vi "RemoteVI Send Overlay.vi"(0 "clients":T2(array[cluster]), 1 "state":T1, 2 "period":dbl=50.0, 5 "overlay popups":T4(array[cluster]), 7 "geo":T3, 9 "d":cluster{"dx":i32, "dy":i32}) -> (4 "clients out":T2(array[cluster]), 6 "state out":T1)   [LabVIEW 2020, in "RemoteVI.lvlib"]
doc: "The OVERLAY part of one server loop iteration (docs\\protocol.md section 3.2). While a popup is open or one was (state.message not empty, to clear it), at most every period ms and only while a client is connected, each popup is captured and PNG-encoded at its LOGICAL position = window position minus (frame origin + d), NOT clipped to the panel, bottom-most first (RemoteVI Encode Popups.vi); RemoteVI Overlay Encode.vi builds the message and it is written to every client (RemoteVI Write To Clients.vi, 500 ms) only when it differs from state.message - an empty OVERLAY when the last popup has closed. state holds the last message, the last frame (sent to a client that connects while a popup is open) - both reset to empty once no popup is open - and the tick count of the last check."
uses:
  RemoteVI.lvlib
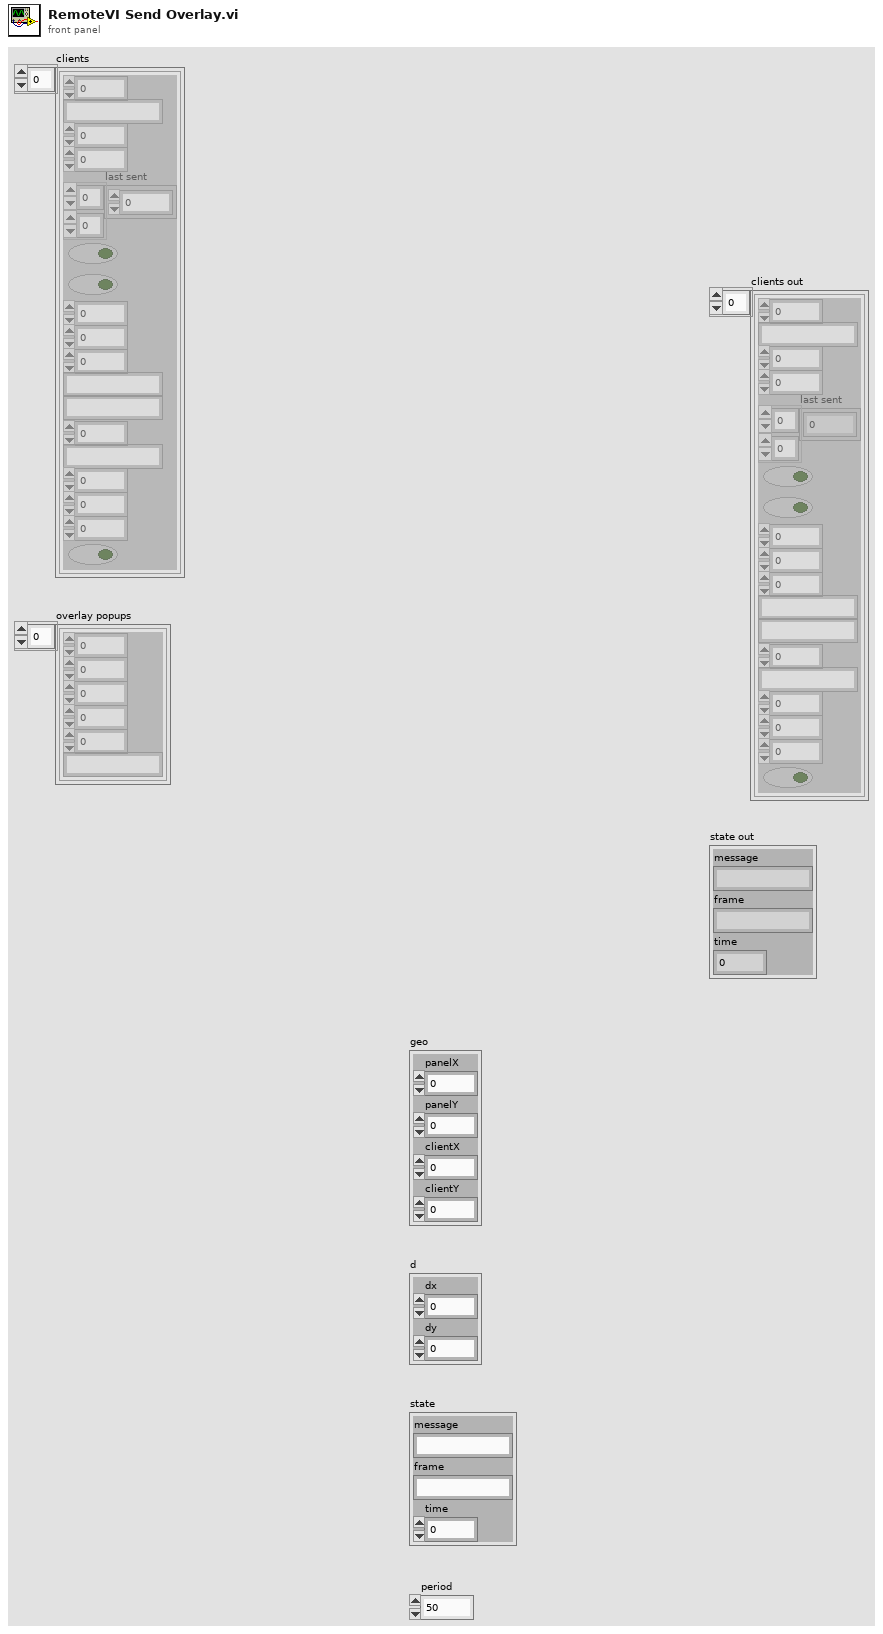
[diagram p1: front panel]
types:
  T1 = cluster{"message":string, "frame":string, "time":u32}
  T2 = cluster{"connection":u32, "rx buffer":string, "seq":u32, "acked":u32, "last sent":u32[][], "tracking":bool, "closed":bool, "mods":u8, "mods set":u8, "popup since":u32, "windows sent":string, "window frames":cluster{"id":u64, "pixels":u32[][]}[], "key window":u64, "address":string, "since":dbl, "last input":dbl, "bytes":dbl, "view only":bool}[]
  T3 = cluster{"panelX":i32, "panelY":i32, "clientX":i32, "clientY":i32}
  T4 = cluster{"hwnd":u64, "x":i32, "y":i32, "w":i32, "h":i32, "class":string}[]
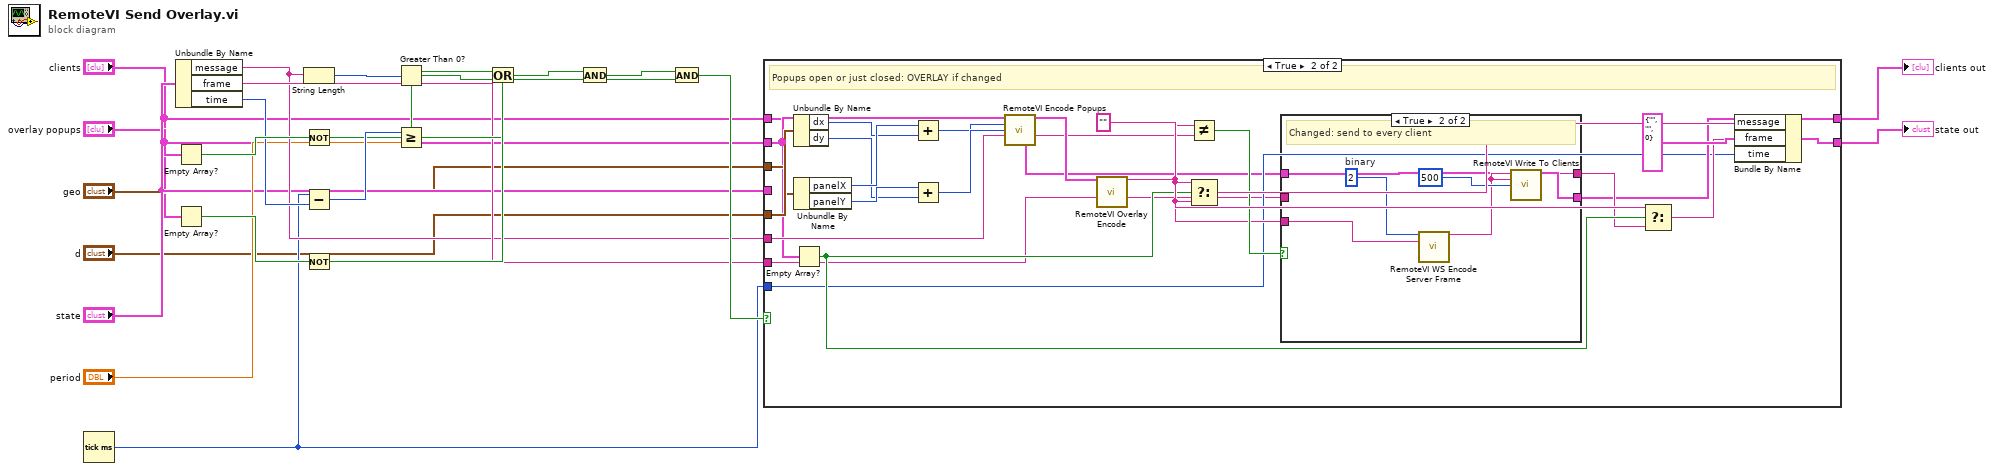
[diagram p0: block diagram]
diagram:
  n1 = Tick Count (ms)() -> (millisecond timer value=w7:u32)
  n2 = Unbundle By Name("state") -> ("message"=w8:string, "frame"=w9:string, "time"=w10:u32)
  n3 = Empty Array?(array="overlay popups") -> (empty?=w13:bool)
  n4 = Empty Array?(array="clients") -> (empty?=w18:bool)
  n5 = String Length(string=w8) -> (length=w11:i32)
  n6 = Not(x=w13) -> (.not. x?=w14:bool)
  n7 = Subtract(x=w7, y=w10) -> (x-y=w16:u32)
  n8 = Not(x=w18) -> (.not. x?=w19:bool)
  n9 = Greater Than 0?(x=w11) -> (x > 0?=w12:bool)
  n10 = Greater Or Equal?(x=w16, y="period") -> (x >= y?=w17:bool)
  n11 = Or(x=w14, y=w12) -> (x .or. y?=w15:bool)
  n12 = And(x=w15, y=w17) -> (x .and. y?=w20:bool)
  n13 = And(x=w20, y=w19) -> (x .and. y?=w21:bool)
  n14 = case shown="True" w21 {
    tunnel: "clients" -> [w24 w26]
    tunnel: "overlay popups" -> [_ w27]
    tunnel: "geo" -> [_ w28]
    tunnel: "state" -> [w25 _]
    tunnel: "d" -> [_ w32]
    tunnel: w8 -> [_ w29]
    tunnel: w9 -> [_ w30]
    tunnel: w7 -> [_ w31]
    tunnel: [w24 w42] -> w22
    tunnel: [w25 w49] -> w23
    frame False {
    }
    frame True {
      w45 = ""
      # "Popups open or just closed: OVERLAY if changed"
      n15 = Unbundle By Name(w32) -> ("dx"=w33:i32, "dy"=w34:i32)
      n16 = Unbundle By Name(w28) -> ("panelX"=w35:i32, "panelY"=w36:i32)
      n17 = Empty Array?(array=w27) -> (empty?=w44:bool)
      n18 = Add(x=w35, y=w33) -> (x+y=w37:i32)
      n19 = Add(x=w36, y=w34) -> (x+y=w38:i32)
      n20 = call "RemoteVI Encode Popups.vi"("popups"=w27, "origin x"=w37, "origin y"=w38) -> ("overlay popups"=w39:cluster{"x":i16, "y":i16, "png":string}[])  [unwired: 12 in]
      n21 = call "RemoteVI Overlay Encode.vi"("popups"=w39) -> ("message"=w40:string)  [unwired: 14 in]
      n22 = Not Equal?(x=w40, y=w29) -> (x != y?=w41:bool)
      n23 = Select(t=w45, s=w44, f=w40) -> (s? t:f=w46:string)
      n24 = case shown="True" w41 {
        tunnel: w26 -> [w50 w52]
        tunnel: w30 -> [w51 _]
        tunnel: w40 -> [_ w53]
        tunnel: [w51 w55] -> w43
        tunnel: [w50 w57] -> w42
        frame False {
        }
        frame True {
          w54 = u8 2  # binary
          # "Changed: send to every client"
          n25 = call "RemoteVI WS Encode Server Frame.vi"("opcode"=w54, "payload"=w53) -> ("frame"=w55:string)  [unwired: 13 in]
          n26 = call "RemoteVI Write To Clients.vi"("clients"=w52, "data"=w55, "timeout ms"=500) -> ("clients out"=w57:T2)  [unwired: 12 in]
        }
      }
      n27 = Select(t=w45, s=w44, f=w43) -> (s? t:f=w47:string)
      n28 = Bundle By Name(cluster=T1 {"message"="", "frame"="", "time"=0}, "message"=w46, "frame"=w47, "time"=w31) -> (w49:T1)
    }
  }
  "clients out" <- w22
  "state out" <- w23
